vi "To XML.vi"(8 "error in (no error)":errorcluster, 9 "Parent":refnum<k20>, 10 "Document":refnum<k20>, 11 "Method in":refnum<class "Method.lvclass">) -> (0 "error out":errorcluster)   [LabVIEW 2017, in "Cobertura.lvlib" / "Method.lvclass"]
uses:
  Method.lvclass
  Method.lvclass/Method.ctl
  <vilib>/xml/Close Reference(Node).vi
  Line/Line.lvclass
  <resource>/objmgr/DOMUserDefRef.rc
  <vilib>/xml/NI_XML.lvlib
  Cobertura.lvlib
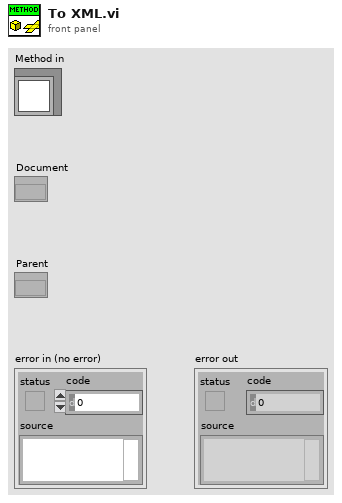
[diagram p1: front panel]
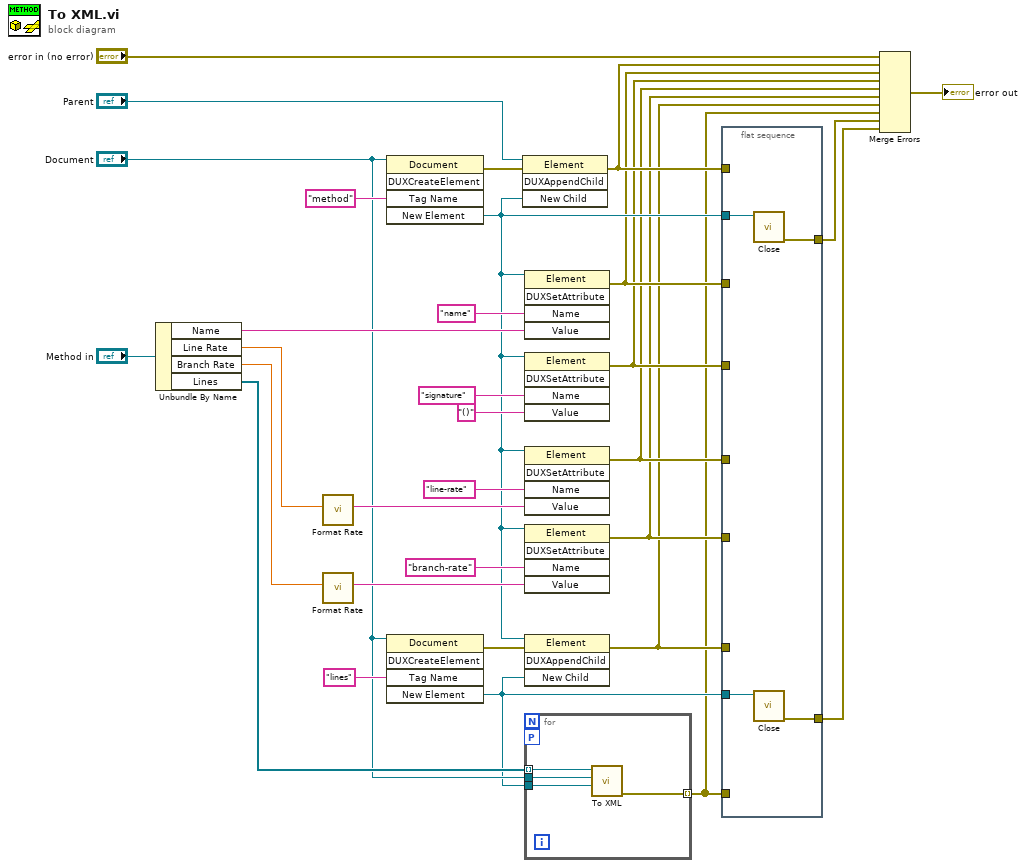
[diagram p0: block diagram]
diagram:
  n1 = Unbundle By Name("Method in") -> ("Name"=w21:string, "Line Rate"=w1:dbl, "Branch Rate"=w2:dbl, "Lines"=w19:refnum<class "Line.lvclass">[])
  n2 = call "Format Rate.vi"("Rate"=w1) -> ("String"=w29:string)  [unwired: 10 in]
  n3 = call "Format Rate.vi"("Rate"=w2) -> ("String"=w27:string)  [unwired: 10 in]
  n4 = invoke class="Document" method="DUXCreateElement"(reference="Document", "Tag Name"="method") -> (error out=w16:errorcluster, "New Element"=w15:refnum<k20>)  [unwired: 3 in, 3 out]
  n5 = invoke class="Document" method="DUXCreateElement"(reference="Document", "Tag Name"="lines") -> (error out=w17:errorcluster, "New Element"=w14:refnum<k20>)  [unwired: 3 in, 3 out]
  n6 = invoke class="Element" method="DUXAppendChild"(reference="Parent", error in=w16, "New Child"=w15) -> (error out=w13:errorcluster)  [unwired: 1 in, 3 out]
  n7 = invoke class="Element" method="DUXSetAttribute"(reference=w15, "Name"="name", "Value"=w21) -> (error out=w12:errorcluster)  [unwired: 2 in, 4 out]
  n8 = invoke class="Element" method="DUXSetAttribute"(reference=w15, "Name"="signature", "Value"="()") -> (error out=w11:errorcluster)  [unwired: 2 in, 4 out]
  n9 = invoke class="Element" method="DUXSetAttribute"(reference=w15, "Name"="line-rate", "Value"=w29) -> (error out=w10:errorcluster)  [unwired: 2 in, 4 out]
  n10 = invoke class="Element" method="DUXSetAttribute"(reference=w15, "Name"="branch-rate", "Value"=w27) -> (error out=w9:errorcluster)  [unwired: 2 in, 4 out]
  n11 = invoke class="Element" method="DUXAppendChild"(reference=w15, error in=w17, "New Child"=w14) -> (error out=w8:errorcluster)  [unwired: 1 in, 3 out]
  n12 = for {
    tunnel: w19 -> [w35] mode=indexing
    tunnel: "Document" -> [w34]
    tunnel: w14 -> [w33]
    workers-P: _ -> [_]
    tunnel: [w32] -> w7 mode=indexing
    n13 = call-dynamic "To XML.vi"("Parent"=w33, "Document"=w34, "Line in"=w35) -> ("error out"=w32:errorcluster)  [unwired: 8 in]
  }
  n14 = flat-sequence {
    tunnel: w15 -> [w39]
    tunnel: w14 -> [w38]
    tunnel: w7 -> [_]
    tunnel: w8 -> [_]
    tunnel: w9 -> [_]
    tunnel: w10 -> [_]
    tunnel: w11 -> [_]
    tunnel: w12 -> [_]
    tunnel: w13 -> [_]
    tunnel: [w37] -> w6
    tunnel: [w36] -> w5
    frame #0 {
      n15 = call-poly <vilib>:"Close.vi"("node"=w39) -> ("error out"=w37:errorcluster)  [unwired: 8 in]
      n16 = call-poly <vilib>:"Close.vi"("node"=w38) -> ("error out"=w36:errorcluster)  [unwired: 8 in]
    }
  }
  n17 = Merge Errors("error in (no error)", w13, w12, w11, w10, w9, w8, w7, w6, w5) -> (→"error out":errorcluster)
